vi "InspectCommandsMac.vi"() -> ()   [LabVIEW 2026]
doc: "Bordeaux: reads one VI's connector, or one control's saved default, in the My Computer context of an already-open project, for the macOS LabVIEW 2026 command catalog. Never runs, edits or saves the VI. Errors: 5101 project not open, 5102 not the My Computer context, 5103 LabVIEW loaded the VI from another path. A blank vi path checks only the project and context."
uses:
  <vilib>/numeric/LVNumericRepresentation.ctl
  <vilib>/Utility/miscctls.llb/LVExtendedInformationArrayTypeDef.ctl
panel:
  out "error out":errorcluster
  out "Modifications After Error":errorcluster
  out "Modifications After:Block Diagram Mods Bitset":u32
  out "Modifications After:Front Panel Mods Bitset":u32
  out "Modifications After:VI Modifications Bitset":u64
  out "Control Value:Get Default":variant
  out "Extended Information":T1
  out "ConNum":u8[](array[numeric])
  out "Data Types":string[](array[string])
  out "I/O Status":u8[](array[numeric])
  out "Wire Requirements":u8[](array[numeric])
  out "Captions":string[](array[string])
  out "Num Connections":u8
  out "Execution:State":T3(ring)
  out "VI Description":string
  out "VI Name":string
  out "VI Type":T4(ring)
  out "VI Path":path
  out "Modifications Error":errorcluster
  out "Modifications:Block Diagram Mods Bitset":u32
  out "Modifications:Front Panel Mods Bitset":u32
  out "Modifications:VI Modifications Bitset":u64
  out "Application:Version Number":string
  out "Application:Context Name":string
  in  "read default":bool
  in  "control name":string
  in  "vi path":string
  in  "project path":string
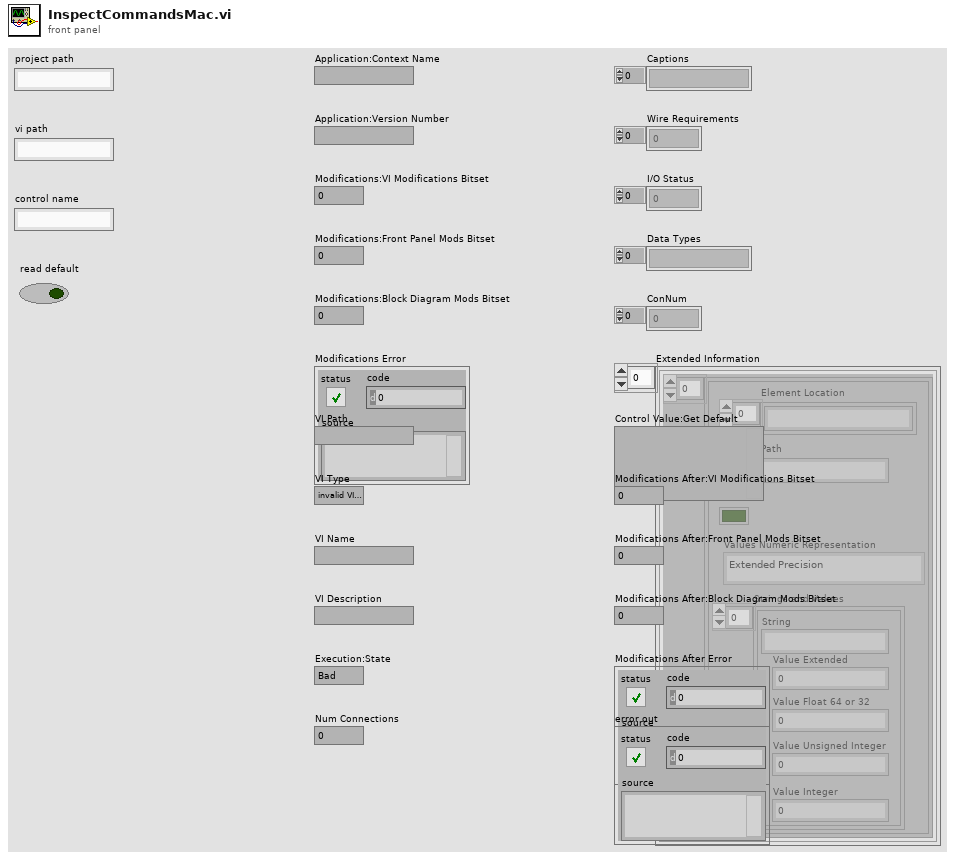
[diagram p1: front panel]
types:
  T1 = typedef "LVExtendedInformationArrayTypeDef.ctl" = cluster{"Extended Data []":cluster{"Element Location":string[], "Typedef Path":path, "Is Enum?":bool, "Values Numeric Representation":T2, "Strings and Values":cluster{"String":string, "Value Extended":ext, "Value Float 64 or 32":dbl, "Value Unsigned Integer":u64, "Value Integer":i64}[]}[]}[]
  T2 = typedef "LVNumericRepresentation.ctl" = enum32{"Extended Precision", "Double Precision", "Single Precision", "Long", "Word", "Byte", "Unsigned Long", "Unsigned Word", "Unsigned Byte", "Complex Extended", "Complex Double", "Complex Single", "Quad", "Unsigned Quad", "Fixed-Point"}
  T3 = enum32{"Bad", "Idle", "Run top level", "Running"}
  T4 = enum32{"invalid VI type", "Standard VI", "Control VI", "Global VI", "Polymorphic VI", "Configuration VI", "SubSystem", "Facade VI", "Method VI", "Statechart Diagram VI"}
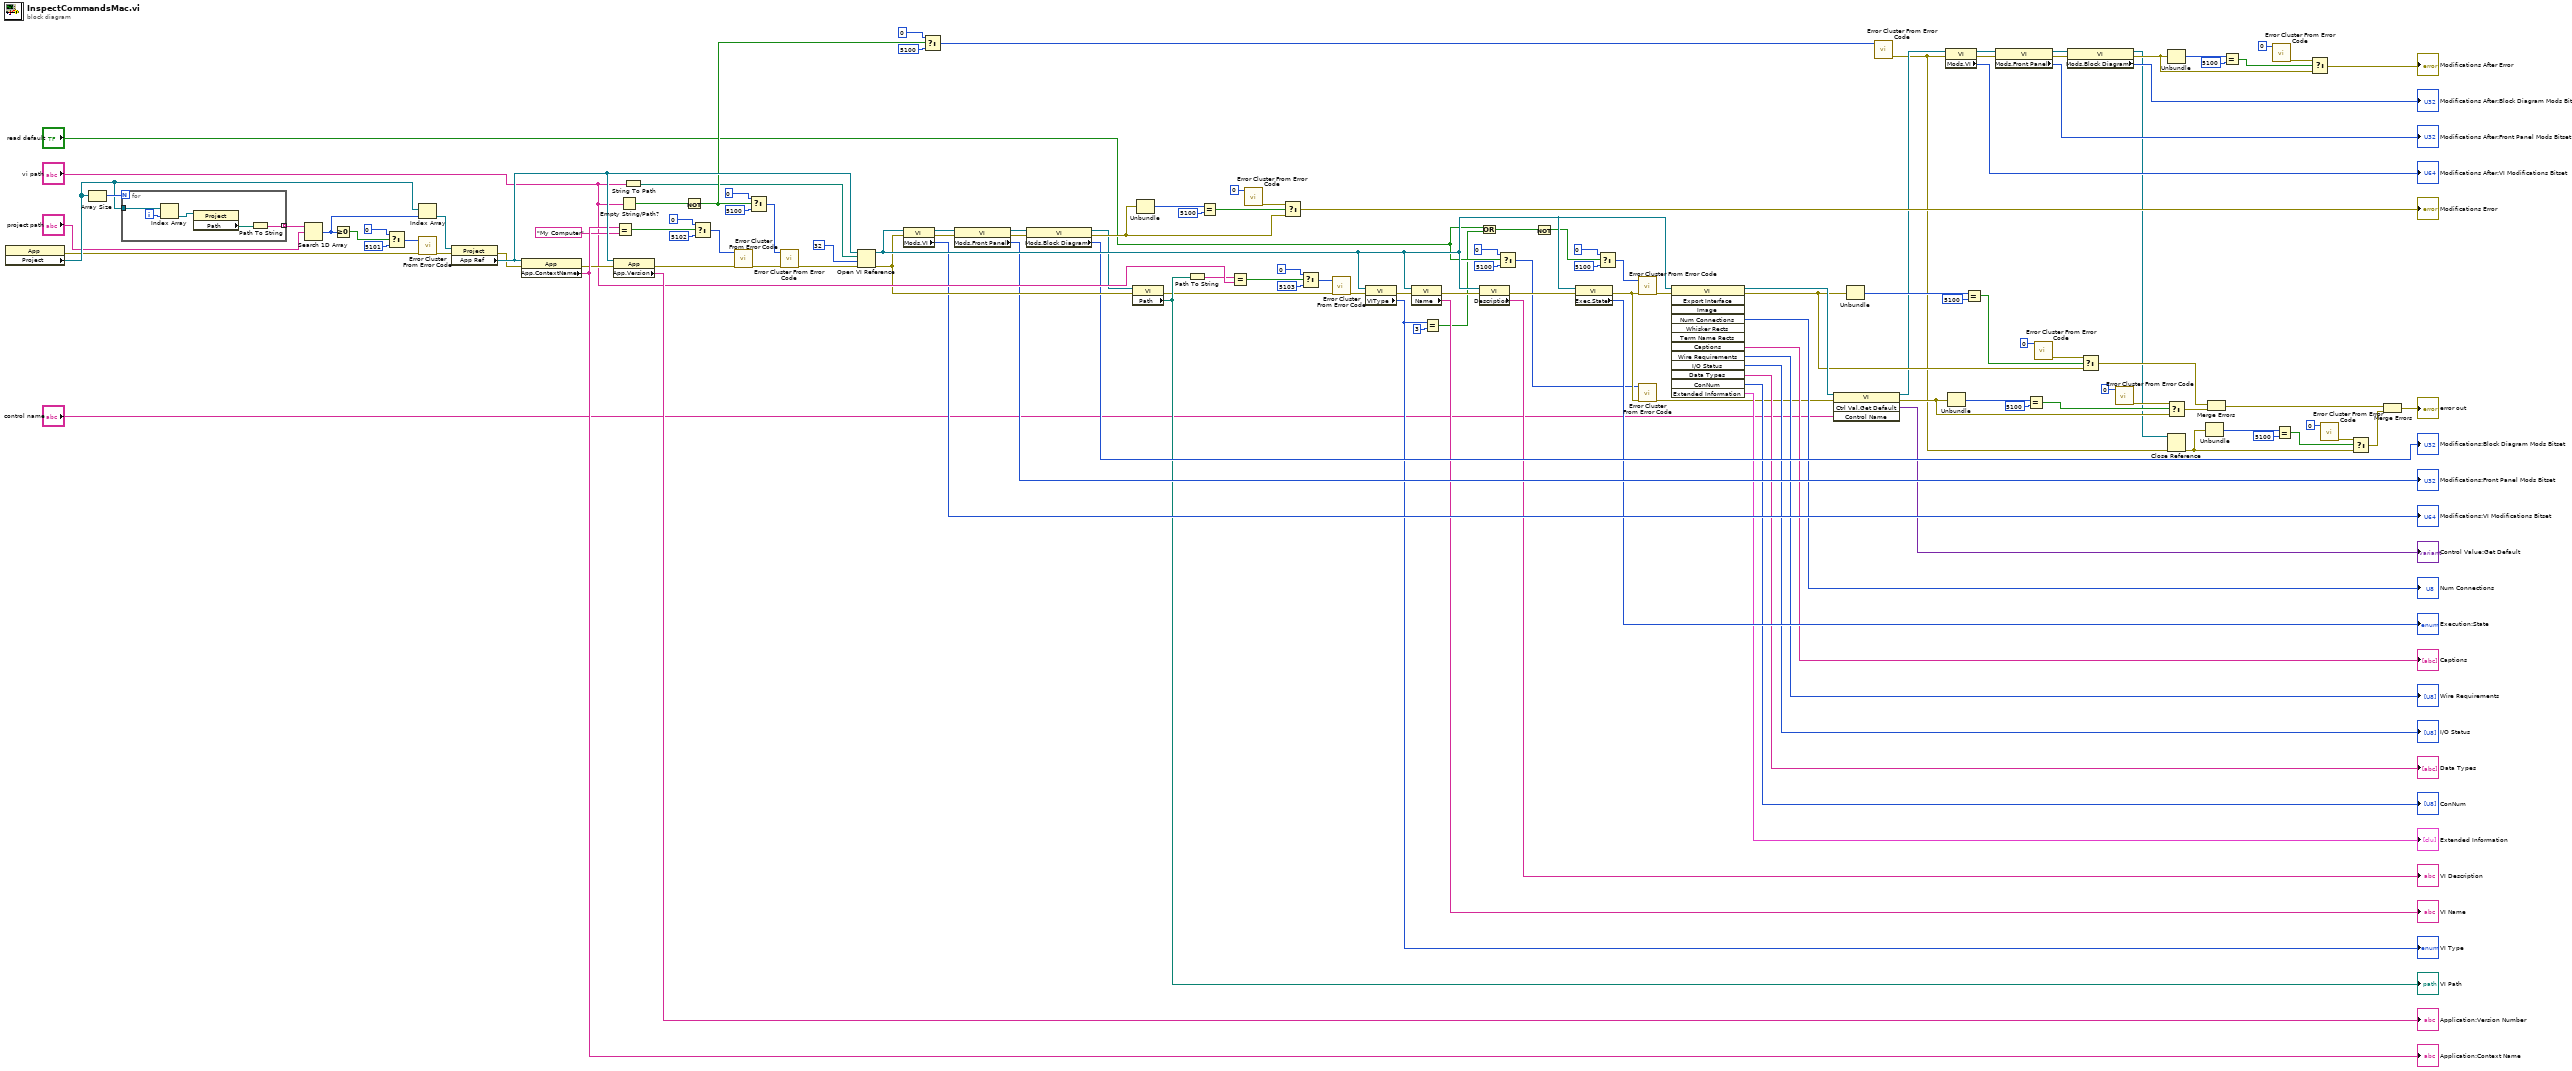
[diagram p0: block diagram]
diagram:
  n1 = property class="App"() -> (error out=w123:errorcluster, "Project"=w131:refnum<vi>[])  [unwired: 2 in, 1 out]
  n2 = Array Size(array=w131) -> (size(s)=w132:i32)
  n3 = for {
    N: w132 -> [_]
    tunnel: w131 -> [w137]
    tunnel: [w133] -> w129 mode=indexing
    i -> [w136]
    n4 = Index Array(array=w137, index=w136) -> (element=w135:refnum<vi>)
    n5 = property class="Project"(reference=w135) -> ("Path"=w134:path)  [unwired: 1 in, 2 out]
    n6 = Path To String(path=w134) -> (string=w133:string)
  }
  n7 = Search 1D Array(1D array=w129, element="project path") -> (index of element=w128:i32)  [unwired: 1 in]
  n8 = Greater Or Equal To 0?(x=w128) -> (x >= 0?=w127:bool)
  n9 = Select(t=0, s=w127, f=5101) -> (s? t:f=w124:i32)
  n10 = Index Array(array=w131, index=w128) -> (element=w122:refnum<vi>)
  n11 = call <vilib>:"Error Cluster From Error Code.vi"("error in (no error)"=w123, "error code (0)"=w124) -> ("error out"=w121:errorcluster)  [unwired: 7 in]
  n12 = property class="Project"(reference=w122, error in=w121) -> (error out=w119:errorcluster, "App Ref"=w120:refnum<vi>)  [unwired: 1 out]
  n13 = property class="App"(reference=w120, error in=w119) -> (error out=w117:errorcluster, "App.ContextName"=w118:string)  [unwired: 1 out]
  "Application:Context Name" <- w118
  n14 = property class="App"(reference=w120, error in=w117) -> (error out=w110:errorcluster, "App.Version"=→"Application:Version Number":string)  [unwired: 1 out]
  n15 = Equal?(x=w118, y="My Computer") -> (x = y?=w114:bool)
  n16 = Empty String/Path?(string/path="vi path") -> (empty?=w108:bool)
  n17 = String To Path(string="vi path") -> (path=w102:path)
  n18 = Not(x=w108) -> (.not. x?=w107:bool)
  n19 = Select(t=0, s=w114, f=5102) -> (s? t:f=w111:i32)
  n20 = call <vilib>:"Error Cluster From Error Code.vi"("error in (no error)"=w110, "error code (0)"=w111) -> ("error out"=w103:errorcluster)  [unwired: 7 in]
  n21 = Select(t=0, s=w107, f=5100) -> (s? t:f=w104:i32)
  n22 = call <vilib>:"Error Cluster From Error Code.vi"("error in (no error)"=w103, "error code (0)"=w104) -> ("error out"=w100:errorcluster)  [unwired: 7 in]
  n23 = Open VI Reference(application reference (local)=w120, vi path=w102, options=u32 32, error in (no error)=w100) -> (vi reference=w99:refnum<vi>, error out=w98:errorcluster)  [unwired: 2 in]
  n24 = property class="VI"(reference=w99, error in=w98) -> (reference out=w96:refnum<vi>, error out=w95:errorcluster, "Mods.VI"=→"Modifications:VI Modifications Bitset":u64)
  n25 = Select(t=0, s=w107, f=5100) -> (s? t:f=w27:i32)
  n26 = property class="VI"(reference=w96, error in=w95) -> (reference out=w93:refnum<vi>, error out=w92:errorcluster, "Mods.Front Panel"=→"Modifications:Front Panel Mods Bitset":u32)
  n27 = property class="VI"(reference=w93, error in=w92) -> (reference out=w83:refnum<vi>, error out=w90:errorcluster, "Mods.Block Diagram"=→"Modifications:Block Diagram Mods Bitset":u32)
  n28 = property class="VI"(reference=w83, error in=w98) -> (error out=w76:errorcluster, "Path"=w82:path)  [unwired: 1 out]
  "VI Path" <- w82
  n29 = Unbundle(w90) -> ("code"=w89:i32)  [unwired: 2 out]
  n30 = Path To String(path=w82) -> (string=w81:string)
  n31 = Equal?(x=w89, y=5100) -> (x = y?=w86:bool)
  n32 = Equal?(x=w81, y="vi path") -> (x = y?=w80:bool)
  n33 = call <vilib>:"Error Cluster From Error Code.vi"("error code (0)"=0) -> ("error out"=w85:errorcluster)  [unwired: 8 in]
  n34 = Select(t=w85, s=w86, f=w90) -> (s? t:f=→"Modifications Error":errorcluster)
  n35 = Select(t=0, s=w80, f=5103) -> (s? t:f=w77:i32)
  n36 = call <vilib>:"Error Cluster From Error Code.vi"("error in (no error)"=w76, "error code (0)"=w77) -> ("error out"=w75:errorcluster)  [unwired: 7 in]
  n37 = property class="VI"(reference=w99, error in=w75) -> (error out=w73:errorcluster, "VIType"=w74:T4)  [unwired: 1 out]
  "VI Type" <- w74
  n38 = property class="VI"(reference=w99, error in=w73) -> (error out=w71:errorcluster, "Name"=→"VI Name":string)  [unwired: 1 out]
  n39 = Equal?(x=w74, y=3) -> (x = y?=w65:bool)
  n40 = property class="VI"(reference=w99, error in=w71) -> (error out=w69:errorcluster, "Description"=→"VI Description":string)  [unwired: 1 out]
  n41 = Or(x="read default", y=w65) -> (x .or. y?=w64:bool)
  n42 = Select(t=0, s="read default", f=5100) -> (s? t:f=w48:i32)
  n43 = Not(x=w64) -> (.not. x?=w63:bool)
  n44 = property class="VI"(reference=w99, error in=w69) -> (error out=w59:errorcluster, "Exec.State"=→"Execution:State":T3)  [unwired: 1 out]
  n45 = Select(t=0, s=w63, f=5100) -> (s? t:f=w60:i32)
  n46 = call <vilib>:"Error Cluster From Error Code.vi"("error in (no error)"=w59, "error code (0)"=w60) -> ("error out"=w58:errorcluster)  [unwired: 7 in]
  n47 = call <vilib>:"Error Cluster From Error Code.vi"("error in (no error)"=w59, "error code (0)"=w48) -> ("error out"=w46:errorcluster)  [unwired: 7 in]
  n48 = invoke class="VI" method="Export Interface"(reference=w99, error in=w58) -> (reference out=w47:refnum<vi>, error out=w43:errorcluster, "Num Connections"=→"Num Connections":u8, "Captions"=→"Captions":string[], "Wire Requirements"=→"Wire Requirements":u8[], "I/O Status"=→"I/O Status":u8[], "Data Types"=→"Data Types":string[], "ConNum"=→"ConNum":u8[], "Extended Information"=→"Extended Information":T1)  [unwired: 11 in, 4 out]
  n49 = invoke class="VI" method="Ctrl Val.Get Default"(reference=w47, error in=w46, "Control Name"="control name") -> (reference out=w26:refnum<vi>, error out=w37:errorcluster, "Ctrl Val.Get Default"=→"Control Value:Get Default":variant)  [unwired: 1 in, 1 out]
  n50 = Unbundle(w43) -> ("code"=w42:i32)  [unwired: 2 out]
  n51 = call <vilib>:"Error Cluster From Error Code.vi"("error code (0)"=w27) -> ("error out"=w25:errorcluster)  [unwired: 8 in]
  n52 = property class="VI"(reference=w26, error in=w25) -> (reference out=w23:refnum<vi>, error out=w22:errorcluster, "Mods.VI"=→"Modifications After:VI Modifications Bitset":u64)
  n53 = Unbundle(w37) -> ("code"=w36:i32)  [unwired: 2 out]
  n54 = Equal?(x=w42, y=5100) -> (x = y?=w39:bool)
  n55 = property class="VI"(reference=w23, error in=w22) -> (reference out=w20:refnum<vi>, error out=w19:errorcluster, "Mods.Front Panel"=→"Modifications After:Front Panel Mods Bitset":u32)
  n56 = Equal?(x=w36, y=5100) -> (x = y?=w33:bool)
  n57 = call <vilib>:"Error Cluster From Error Code.vi"("error code (0)"=0) -> ("error out"=w38:errorcluster)  [unwired: 8 in]
  n58 = property class="VI"(reference=w20, error in=w19) -> (reference out=w10:refnum<vi>, error out=w17:errorcluster, "Mods.Block Diagram"=→"Modifications After:Block Diagram Mods Bitset":u32)
  n59 = Select(t=w38, s=w39, f=w43) -> (s? t:f=w31:errorcluster)
  n60 = call <vilib>:"Error Cluster From Error Code.vi"("error code (0)"=0) -> ("error out"=w32:errorcluster)  [unwired: 8 in]
  n61 = Unbundle(w17) -> ("code"=w16:i32)  [unwired: 2 out]
  n62 = Select(t=w32, s=w33, f=w37) -> (s? t:f=w30:errorcluster)
  n63 = Close Reference(reference=w10, error in (no error)=w25) -> (error out=w9:errorcluster)
  n64 = Unbundle(w9) -> ("code"=w8:i32)  [unwired: 2 out]
  n65 = Merge Errors(w31, w30) -> (w3:errorcluster)
  n66 = Equal?(x=w16, y=5100) -> (x = y?=w13:bool)
  n67 = call <vilib>:"Error Cluster From Error Code.vi"("error code (0)"=0) -> ("error out"=w12:errorcluster)  [unwired: 8 in]
  n68 = Equal?(x=w8, y=5100) -> (x = y?=w5:bool)
  n69 = Select(t=w12, s=w13, f=w17) -> (s? t:f=→"Modifications After Error":errorcluster)
  n70 = call <vilib>:"Error Cluster From Error Code.vi"("error code (0)"=0) -> ("error out"=w4:errorcluster)  [unwired: 8 in]
  n71 = Select(t=w4, s=w5, f=w9) -> (s? t:f=w2:errorcluster)
  n72 = Merge Errors(w3, w2) -> (→"error out":errorcluster)
